vi "ZM-PC-init.vi"(8 "error in (no error)":errorcluster, 11 "ZM-PC-TP-test_package in":refnum<class "ZM-PC-TP-test_package.lvclass">) -> (0 "error out":errorcluster, 3 "ZM-PC-TP-test_package out":refnum<class "ZM-PC-TP-test_package.lvclass">)   [LabVIEW 2020, in "ZM-PC-packages.lvlib" / "ZM-PC-TP-test_package.lvclass"]
doc: "Initialises a package (dynamic dispatch): writes the current time from Get Date/Time In Seconds through Write timestamp and the type Undefined through Write type. The destination is not touched. Each child overrides it with Call Parent followed by its own setType hook."
uses:
  ZM-PC-TP-test_package.lvclass
  ZM-PC-package/ZM-PC-package.lvclass
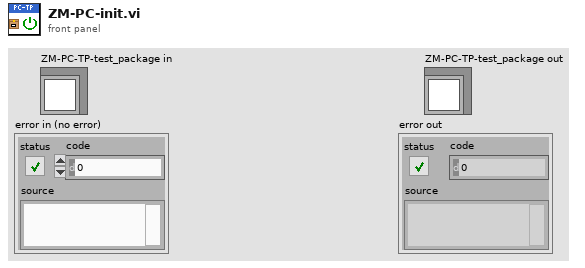
[diagram p1: front panel]
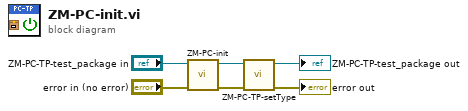
[diagram p0: block diagram]
diagram:
  n1 = call-parent "ZM-PC-init.vi"("error in (no error)"="error in (no error)", "ZM-PC-package in"="ZM-PC-TP-test_package in") -> ("error out"=w1:errorcluster, "ZM-PC-package out"=w3:refnum<class "ZM-PC-TP-test_package.lvclass">)  [unwired: 8 in]
  n2 = call "ZM-PC-TP-setType.vi"("error in (no error)"=w1, "ZM-PC-package in"=w3) -> ("error out"=→"error out":errorcluster, "ZM-PC-package out"=→"ZM-PC-TP-test_package out":refnum<class "ZM-PC-TP-test_package.lvclass">)  [unwired: 8 in]
